vi "RemoteVI Dirty Band.vi"(0 "previous":u32[][](array[numeric]), 1 "tile size":i32=64, 2 "width":i32, 5 "current":u32[][](array[numeric]), 7 "y":i32, 9 "h":i32) -> (4 "x":i32, 6 "w":i32)   [LabVIEW 2020, in "RemoteVI.lvlib"]
doc: "The changed part of one tile row (band) of two panel captures: rows y to y + h - 1 are compared tile by tile (tile size x h, tiles clipped at the right edge, every pixel equal - Equal? then And Array Elements). x is the left edge of the first dirty tile, w the distance from there to the right edge of the last dirty tile. Call it only for a band that differs (RemoteVI Dirty Rects.vi does); in a band without a dirty tile x and w are meaningless. Pure and reentrant."
uses:
  RemoteVI.lvlib
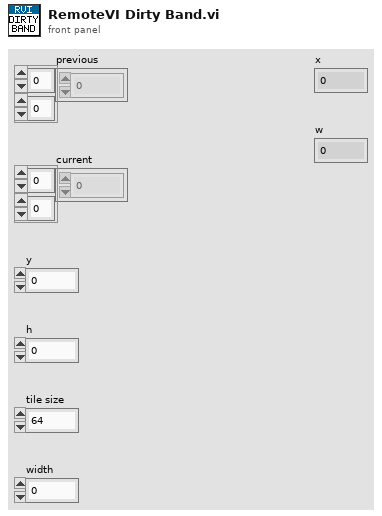
[diagram p1: front panel]
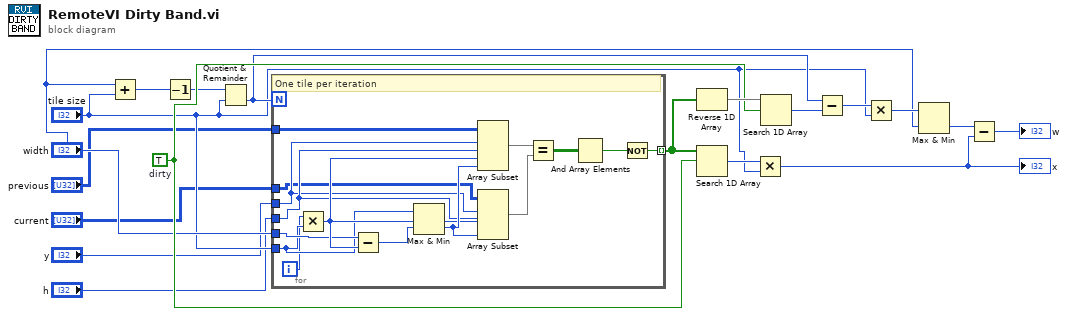
[diagram p0: block diagram]
diagram:
  w11 = TRUE  # dirty
  n1 = Add(x="width", y="tile size") -> (x+y=w7:i32)
  n2 = Decrement(x=w7) -> (x-1=w8:i32)
  n3 = Quotient & Remainder(x=w8, y="tile size") -> (floor(x/y)=w9:i32)  [unwired: 1 out]
  n4 = for {
    N: w9 -> [_]
    tunnel: "previous" -> [w21]
    tunnel: "current" -> [w22]
    tunnel: "tile size" -> [w23]
    tunnel: "width" -> [w24]
    tunnel: "y" -> [w25]
    tunnel: "h" -> [w26]
    tunnel: [w34] -> w10 mode=indexing
    i -> [w20]
    # "One tile per iteration"
    n5 = Multiply(x=w20, y=w23) -> (x*y=w27:i32)
    n6 = Subtract(x=w24, y=w27) -> (x-y=w28:i32)
    n7 = Max & Min(x=w23, y=w28) -> (min(x,y)=w29:i32)  [unwired: 1 out]
    n8 = Array Subset(array=w21, index (row)=w25, length (row)=w26, index (col)=w27, length (col)=w29) -> (w30:u32[][])
    n9 = Array Subset(array=w22, index (row)=w25, length (row)=w26, index (col)=w27, length (col)=w29) -> (w31:u32[][])
    n10 = Equal?(x=w30, y=w31) -> (x = y?=w32:bool[][])
    n11 = And Array Elements(Boolean array=w32) -> (logical AND=w33:bool)
    n12 = Not(x=w33) -> (.not. x?=w34:bool)
  }
  n13 = Reverse 1D Array(array=w10) -> (reversed array=w13:bool[])
  n14 = Search 1D Array(1D array=w10, element=w11) -> (index of element=w12:i32)  [unwired: 1 in]
  n15 = Multiply(x=w12, y="tile size") -> (x*y=w15:i32)
  "x" <- w15
  n16 = Search 1D Array(1D array=w13, element=w11) -> (index of element=w14:i32)  [unwired: 1 in]
  n17 = Subtract(x=w9, y=w14) -> (x-y=w16:i32)
  n18 = Multiply(x=w16, y="tile size") -> (x*y=w17:i32)
  n19 = Max & Min(x=w17, y="width") -> (min(x,y)=w18:i32)  [unwired: 1 out]
  n20 = Subtract(x=w18, y=w15) -> (x-y=→"w":i32)
